vi "onTestExecution.vi"(6 "timeout (2000 ms)":i32=2000, 7 "Name":string, 8 "error in (no error)":errorcluster, 11 "Test Runner.BrokenTests in":refnum<class "Test Runner.BrokenTest.lvclass">) -> (0 "error out":errorcluster, 3 "Test Runner.BrokenTests":refnum<class "Test Runner.BrokenTest.lvclass">)   [LabVIEW 2020, in "Test Runner.BrokenTest.lvclass"]
uses:
  Test Runner.BrokenTest.lvclass
  C:/projects/caraya/src/classes/Test Runner/Test Runner.lvclass
  classes/Test Runner/Test Runner.lvclass/Test Runner.ctl
  classes/Assert/Assert Not Error.vi
  classes/Assert/Assert Error.vi
  classes/Test/Test.lvclass
  classes/Assert/Assert.lvclass
  classes/Test Runner/Test Runner.lvclass
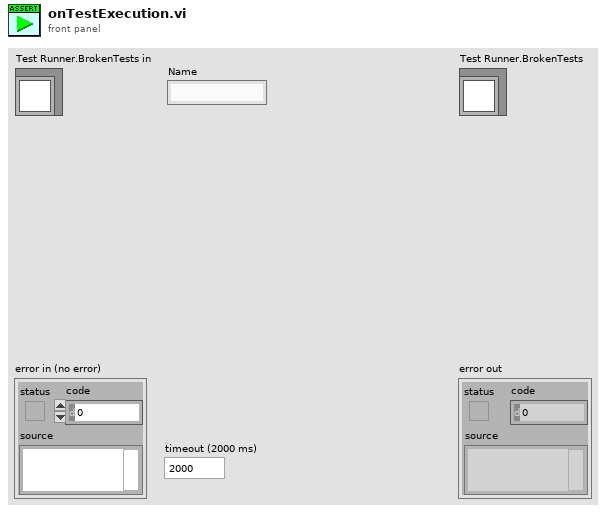
[diagram p1: front panel]
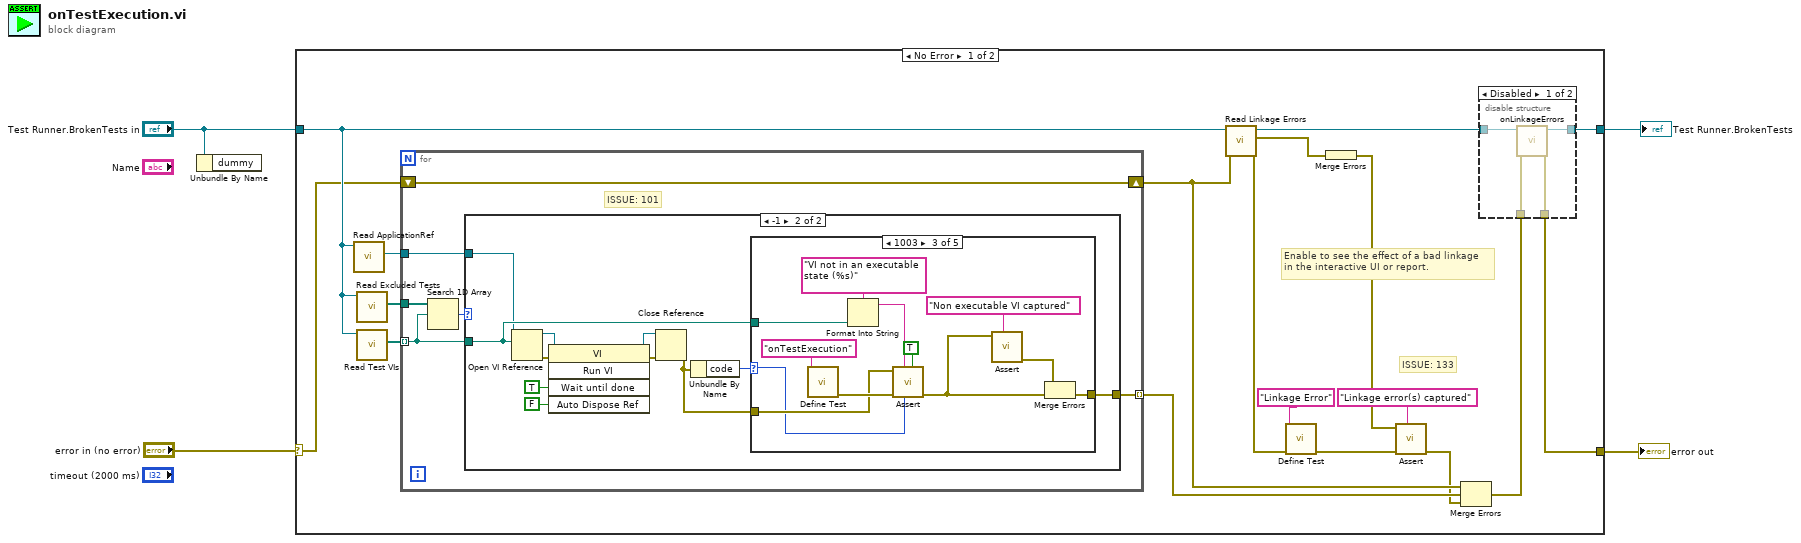
[diagram p0: block diagram]
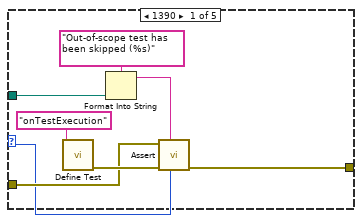
[diagram p4: hidden frame]
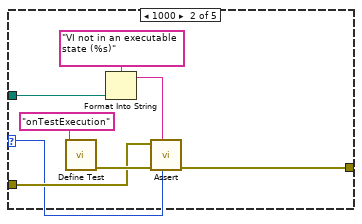
[diagram p5: hidden frame]
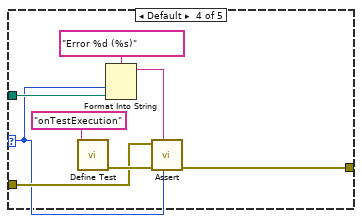
[diagram p6: hidden frame]
diagram:
  n1 = Unbundle By Name("Test Runner.BrokenTests in") -> ()  [unwired: 1 out]
  n2 = case shown="No Error" "error in (no error)" {
    selector: "error in (no error)" -> [w11 w83]
    tunnel: "Test Runner.BrokenTests in" -> [w12 w84]
    tunnel: [w7 w84] -> w3
    tunnel: [w6 w83] -> w1
    frame No Error {
      # "ISSUE: 133"
      # "Enable to see the effect of a bad linkage\nin the interactive UI or report."
      n3 = call "Read ApplicationRef.vi"("Test Runner in"=w12) -> ("Application"=w13:refnum<vi>)  [unwired: 8 in, 2 out]
      n4 = call "Read Excluded Tests.vi"("Test Runner in"=w12) -> ("Excluded Tests"=w15:path[])  [unwired: 8 in, 2 out]
      n5 = call "Read Test VIs.vi"("Test Runner in"=w12) -> ("Test VIs"=w14:path[])  [unwired: 8 in, 2 out]
      n6 = for {
        tunnel: w14 -> [w33] mode=indexing
        tunnel: [w32] -> w16 mode=indexing
        tunnel: w15 -> [w34]
        tunnel: w13 -> [w30]
        shift-right: [w29] -> w10
        shift-left: w11 -> [w29]
        # "ISSUE: 101"
        n7 = Search 1D Array(1D array=w34, element=w33) -> (index of element=w31:i32)  [unwired: 1 in]
        n8 = case shown="-1" w31 {
          tunnel: w33 -> [_ w37]
          tunnel: [_ w36] -> w32
          tunnel: w30 -> [_ w35]
          frame Default {
            # "Test is part of the exclusion list"
          }
          frame -1 {
            n9 = Open VI Reference(application reference (local)=w35, vi path=w37) -> (vi reference=w38:refnum<vi>, error out=w45:errorcluster)  [unwired: 4 in]
            n10 = invoke on="Invoke Node" class="VI" method="Run VI"(reference=w38, error in=w45, "Wait until done"=TRUE ("Wait Until Done"), "Auto Dispose Ref"=FALSE ("Auto Dispose Reference")) -> (reference out=w41:refnum<vi>, error out=w40:errorcluster)  [unwired: 1 in, 3 out]
            n11 = Close Reference(reference=w41, error in (no error)=w40) -> (error out=w39:errorcluster)
            n12 = Unbundle By Name(w39) -> ("code"=w42:i32)
            n13 = case shown="1003" w42 {
              selector: w42 -> [w46 w54 w67 w74 _]
              tunnel: w39 -> [w47 w55 w68 w75 w82]
              tunnel: [w49 w57 w63 w78 w82] -> w36
              tunnel: w37 -> [w53 w61 w73 w81 _]
              frame 1390 {
                n14 = call "Define Test.vi"("Label (VI Title)"="onTestExecution" ("Label")) -> ("error out"=w50:errorcluster)  [unwired: 9 in, 1 out]
                n15 = Format Into String(format string="Out-of-scope test has been skipped (%s)" ("Label"), w53) -> (resulting string=w48:string)  [unwired: 2 in, 1 out]
                n16 = call-poly "Assert.vi"("error code (1)"=w46, "Label"=w48, "error in (no error)"=w50, "Not Error?"=w47) -> ("error out"=w49:errorcluster)  [unwired: 6 in, 1 out]
              }
              frame 1000 {
                n17 = call "Define Test.vi"("Label (VI Title)"="onTestExecution" ("Label")) -> ("error out"=w58:errorcluster)  [unwired: 9 in, 1 out]
                n18 = Format Into String(format string="VI not in an executable state (%s)" ("Label"), w61) -> (resulting string=w56:string)  [unwired: 2 in, 1 out]
                n19 = call-poly "Assert.vi"("error code (1)"=w54, "Label"=w56, "error in (no error)"=w58, "Not Error?"=w55) -> ("error out"=w57:errorcluster)  [unwired: 6 in, 1 out]
              }
              frame 1003 {
                n20 = call "Define Test.vi"("Label (VI Title)"="onTestExecution" ("Label")) -> ("error out"=w70:errorcluster)  [unwired: 9 in, 1 out]
                n21 = Format Into String(format string="VI not in an executable state (%s)" ("Label"), w73) -> (resulting string=w69:string)  [unwired: 2 in, 1 out]
                n22 = call-poly "Assert.vi"("Assert Only? (F)"=TRUE, "error code (1)"=w67, "Label"=w69, "error in (no error)"=w70, "Not Error?"=w68) -> ("error out"=w64:errorcluster)  [unwired: 5 in, 1 out]
                n23 = call-poly "Assert.vi"("Label"="Non executable VI captured", "Error?"=w64) -> ("error out"=w62:errorcluster)  [unwired: 8 in, 1 out]
                n24 = Merge Errors(w62, w64) -> (w63:errorcluster)
              }
              frame Default {
                n25 = call "Define Test.vi"("Label (VI Title)"="onTestExecution" ("Label")) -> ("error out"=w76:errorcluster)  [unwired: 9 in, 1 out]
                n26 = Format Into String(format string="Error %d (%s)" ("Label"), w74, w81) -> (resulting string=w77:string)  [unwired: 2 in, 1 out]
                n27 = call-poly "Assert.vi"("error code (1)"=w74, "Label"=w77, "error in (no error)"=w76, "Not Error?"=w75) -> ("error out"=w78:errorcluster)  [unwired: 6 in, 1 out]
              }
              frame 0 {
              }
            }
          }
        }
      }
      n28 = call "Read Linkage Errors.vi"("error in (no error)"=w10, "Test Runner in"=w12) -> ("error out"=w17:errorcluster, "Linkage Errors"=w19:errorcluster[], "Test Runner out"=w8:refnum<class "Test Runner.BrokenTest.lvclass">)  [unwired: 7 in]
      n29 = call "Define Test.vi"("error in (no error)"=w17, "Label (VI Title)"="Linkage Error" ("Label")) -> ("error out"=w21:errorcluster)  [unwired: 8 in, 1 out]
      n30 = Merge Errors(w19) -> (w18:errorcluster)
      n31 = call-poly "Assert.vi"("Label"="Linkage error(s) captured", "error in (no error)"=w21, "Error?"=w18) -> ("error out"=w9:errorcluster)  [unwired: 7 in, 1 out]
      n32 = Merge Errors(w10, w16, w9) -> (w5:errorcluster)
      n33 = disable-structure "Diagram Disable Structure" shown="Disabled" {
        disable-tunnel: w8 -> [w26 w28]
        disable-tunnel: [w25 w28] -> w7
        disable-tunnel: [w24 w27] -> w6
        disable-tunnel: w5 -> [w23 w27]
        frame Disabled {
          n34 = call-dynamic "onLinkageErrors.vi"("error in (no error)"=w23, "Test Runner in"=w26) -> ("error out"=w24:errorcluster, "Test Runner out"=w25:refnum<class "Test Runner.BrokenTest.lvclass">)  [unwired: 8 in]
        }
        frame Enabled {
        }
      }
    }
    frame Error {
    }
  }
  "error out" <- w1
  "Test Runner.BrokenTests" <- w3
